vi "Read Partial Raw.vi"(8 "error in (no error)":errorcluster, 9 "Read Offset (bytes)":u32, 10 "Data In":u8[](array[numeric]), 11 "Raw Reader Reference":T1 {"refnum" format="%.0x"}) -> (0 "error out":errorcluster, 1 "Data Length":u32, 2 "Data Out":u8[](array[numeric]))   [LabVIEW 2021, in "Iceoryx.lvlib"]
uses:
  Iceoryx.lvlib
  Refnum/Typedef/BB Raw Reader Refnum.ctl
  SubVIs/Convert Error Core.vi
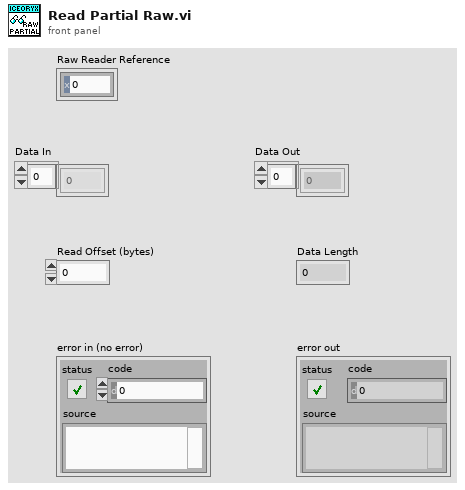
[diagram p1: front panel]
types:
  T1 = typedef "Iceoryx.lvlib/BB Raw Reader Refnum.ctl" = cluster{"refnum":u64, "BB Raw Reader":enum8{"bb_raw_reader"}}
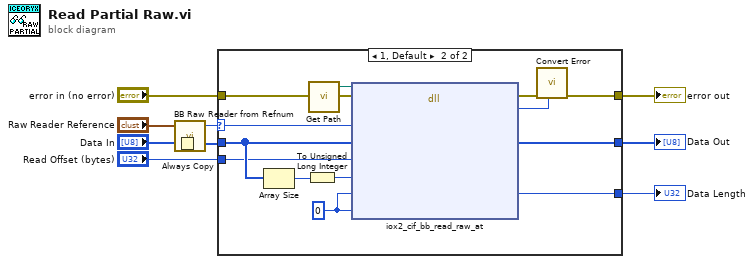
[diagram p0: block diagram]
diagram:
  n1 = Always Copy(1:"Data In") -> (0:w1:u8[])
  n2 = call "BB Raw Reader from Refnum.vi"("BB Raw Reader Refnum"="Raw Reader Reference") -> ("BB Raw Reader U64"=w3:u64)  [unwired: 4 in]
  n3 = case shown="1, Default" w3 {
    selector: w3 -> [_ w19]
    tunnel: "error in (no error)" -> [w11 w24]
    tunnel: w1 -> [w10 w18]
    tunnel: [w10 w14] -> w6
    tunnel: [w11 w20] -> w8
    tunnel: [_ w12] -> w5
    tunnel: "Read Offset (bytes)" -> [_ w13]
    frame 0 {
    }
    frame 1, Default {
      w15 = u32 0 ("actual")
      n4 = Array Size(array=w18) -> (size(s)=w17:i32)
      n5 = To Unsigned Long Integer(number=w17) -> (unsigned 32bit integer=w16:u32)
      n6 = call "Get Path.vi"() -> ("libiox2_cif path"=w23:path)  [unwired: 4 in]
      n7 = dll-call lib="D:/dev/iceoryx2_lvwrapper/dist/iox2_cif.dll" fn="iox2_cif_bb_read_raw_at"(path in=w23, error in=w24, "reader"=w19, "bytes"=w18, "offset_bytes"=w13, "cap_bytes"=w16, "actual_bytes"=w15, "max_bytes"=w15) -> (error out=w22:errorcluster, "return type"=w21:i32, "bytes"=w14:u8[], "actual_bytes"=w12:u32)  [unwired: 5 in, 1 out]
      n8 = call "Convert Error.vi"("return type"=w21, "error in (no error)"=w22) -> ("error out"=w20:errorcluster)  [unwired: 9 in]
    }
  }
  "error out" <- w8
  "Data Out" <- w6
  "Data Length" <- w5
